vi "Write Headline.vi"(9 "other":i32, 10 "stock":i32, 11 "template":string) -> (3 "headline":string)   [LabVIEW 2020, in "Full Featured MCP Server.lvlib"]
doc: "Fills in a headline template: {stock} becomes the name of the stock, {other} the name of the second stock and {sector} the sector of the stock."
uses:
  Full Featured MCP Server.lvlib
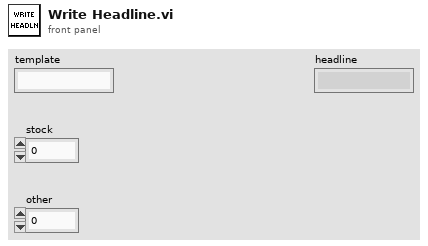
[diagram p1: front panel]
types:
  T1 = cluster{"name":string, "sector":i32, "quality":i32, "start price":dbl, "drift":dbl, "volatility":dbl, "beta":dbl, "jumpiness":dbl, "description":string}[]
  T2 = cluster{"name":string, "sector":i32, "quality":i32, "start price":dbl, "drift":dbl, "volatility":dbl, "beta":dbl, "jumpiness":dbl, "description":string}
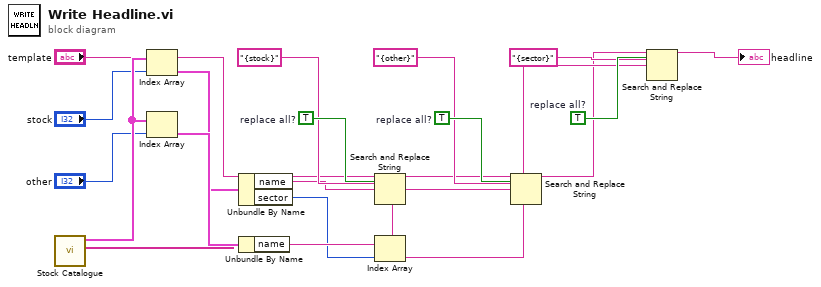
[diagram p0: block diagram]
diagram:
  w19 = TRUE  # replace all?
  w15 = TRUE  # replace all?
  w12 = TRUE  # replace all?
  n1 = call "Stock Catalogue.vi"() -> ("sectors"=w5:string[], "stocks"=w4:T1)  [unwired: 10 in]
  n2 = Index Array(array=w4, index="stock") -> (element=w6:T2)
  n3 = Index Array(array=w4, index="other") -> (element=w9:T2)
  n4 = Unbundle By Name(w6) -> ("name"=w7:string, "sector"=w8:i32)
  n5 = Unbundle By Name(w9) -> ("name"=w10:string)
  n6 = Search and Replace String(replace all?=w12, input string="template", search string="{stock}", replace string=w7) -> (result string=w13:string)  [unwired: 4 in, 3 out]
  n7 = Index Array(array=w5, index=w8) -> (element=w17:string)
  n8 = Search and Replace String(replace all?=w15, input string=w13, search string="{other}", replace string=w10) -> (result string=w16:string)  [unwired: 4 in, 3 out]
  n9 = Search and Replace String(replace all?=w19, input string=w16, search string="{sector}", replace string=w17) -> (result string=→"headline":string)  [unwired: 4 in, 3 out]
